vi "WD_Heartbeat.vi"(8 "error in (no error)":errorcluster, 11 "Stop Queue":refnum<queue>) -> (0 "error out":errorcluster)   [LabVIEW 2018]
doc: "Use this template to build a VI to use as a subVI."
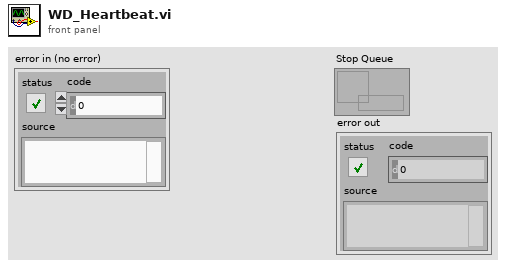
[diagram p1: front panel]
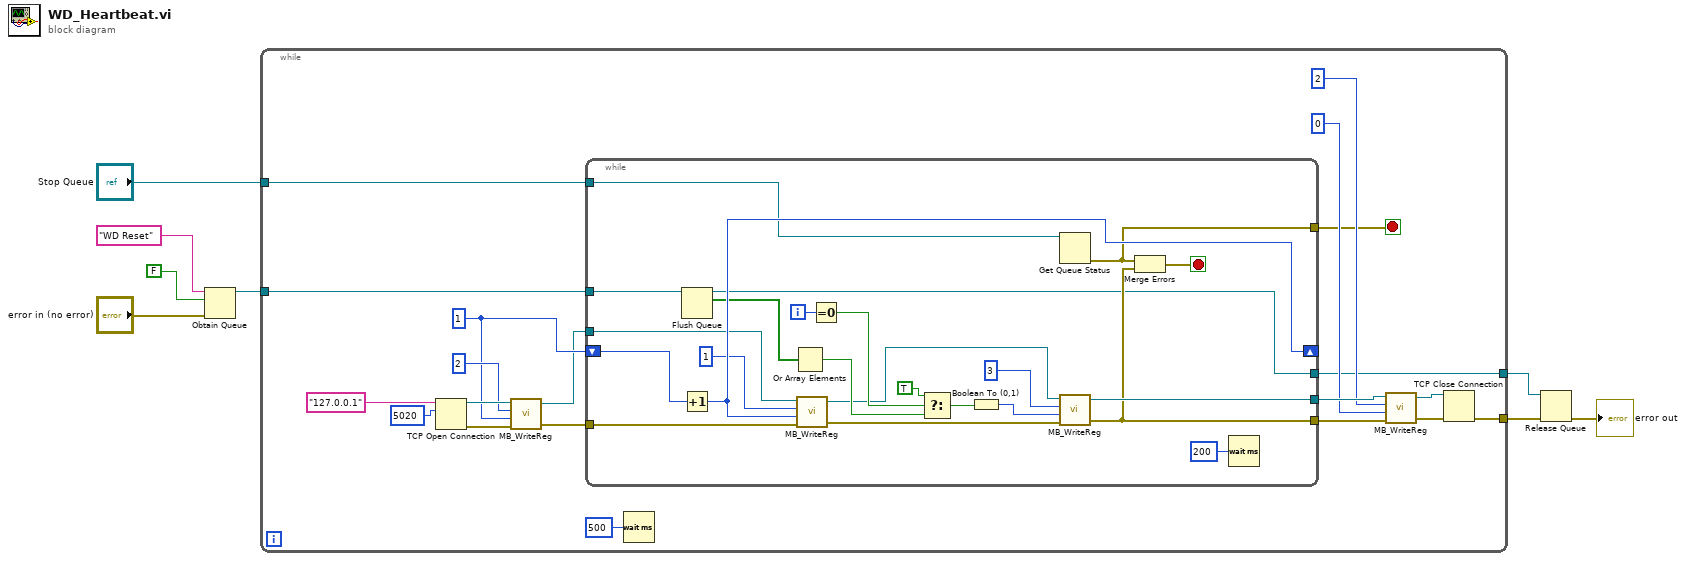
[diagram p0: block diagram]
diagram:
  n1 = Obtain Queue(name (unnamed)="WD Reset", element data type=FALSE, error in (no error)="error in (no error)") -> (queue out=w5:refnum<queue>)  [unwired: 2 in, 2 out]
  n2 = while {
    tunnel: w5 -> [w19]
    tunnel: "Stop Queue" -> [w18]
    tunnel: [w10] -> w3
    tunnel: [w9] -> w2
    stop <- w11 stop-if-true
    w23 = u16 1 ("Value")
    n3 = TCP Open Connection(address="127.0.0.1", remote port or service name=u16 5020) -> (connection ID=w26:refnum<k5>, error out=w25:errorcluster)  [unwired: 3 in]
    n4 = call "MB_WriteReg.vi"("error in (no error)"=w25, "Value"=w23, "Address"=u16 2, "connection ID"=w26) -> ("error out"=w20:errorcluster, "connection ID out"=w21:refnum<k5>)  [unwired: 1 in]
    n5 = while {
      shift-right: [w50] -> _
      shift-left: w23 -> [w51]
      tunnel: w21 -> [w48]
      tunnel: w20 -> [w47]
      tunnel: w19 -> [w46]
      tunnel: w18 -> [w34]
      tunnel: [w32] -> w17
      tunnel: [w31] -> w16
      tunnel: [w30] -> w11
      tunnel: [w29] -> w10
      i -> [w44]
      stop <- w33 stop-if-true
      n6 = Flush Queue(queue=w46) -> (queue out=w29:refnum<queue>, remaining elements=w45:bool[])  [unwired: 1 in, 1 out]
      n7 = Increment(x=w51) -> (x+1=w50:u16)
      n8 = Or Array Elements(Boolean array=w45) -> (logical OR=w41:bool)
      n9 = call "MB_WriteReg.vi"("error in (no error)"=w47, "Value"=w50, "Address"=u16 1, "connection ID"=w48) -> ("error out"=w38:errorcluster, "connection ID out"=w39:refnum<k5>)  [unwired: 1 in]
      n10 = Equal To 0?(x=w44) -> (x = 0?=w43:bool)
      n11 = Select(t=TRUE, s=w43, f=w41) -> (s? t:f=w40:bool)
      n12 = Boolean To (0,1)(Boolean=w40) -> (0, 1=w36:i16)
      n13 = Get Queue Status(queue=w34) -> (error out=w30:errorcluster)  [unwired: 2 in, 7 out]
      n14 = call "MB_WriteReg.vi"("error in (no error)"=w38, "Value"=w36, "Address"=u16 3, "connection ID"=w39) -> ("error out"=w31:errorcluster, "connection ID out"=w32:refnum<k5>)  [unwired: 1 in]
      n15 = Merge Errors(w30, w31) -> (w33:errorcluster)
      n16 = Wait (ms)(milliseconds to wait=u32 200) -> ()  [unwired: 1 out]
    }
    n17 = Wait (ms)(milliseconds to wait=u32 500) -> ()  [unwired: 1 out]
    n18 = call "MB_WriteReg.vi"("error in (no error)"=w16, "Value"=u16 0, "Address"=u16 2, "connection ID"=w17) -> ("error out"=w12:errorcluster, "connection ID out"=w13:refnum<k5>)  [unwired: 1 in]
    n19 = TCP Close Connection(connection ID=w13, error in (no error)=w12) -> (error out=w9:errorcluster)  [unwired: 1 in, 1 out]
  }
  n20 = Release Queue(queue=w3, error in (no error)=w2) -> (error out=→"error out":errorcluster)  [unwired: 1 in, 2 out]
